vi "Test Li.vi"() -> ()   [LabVIEW 2026]
panel:
  out "XY Graph":cluster{dbl[], dbl[]}[](graph)
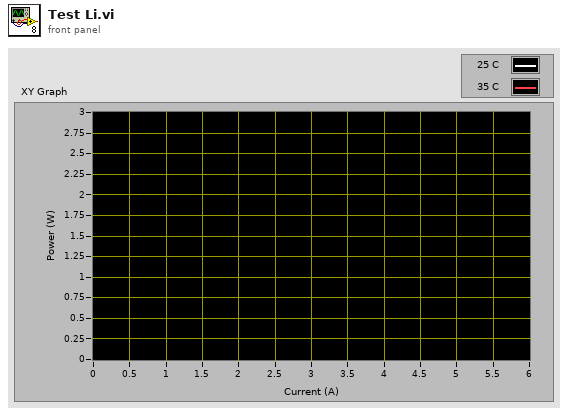
[diagram p1: front panel]
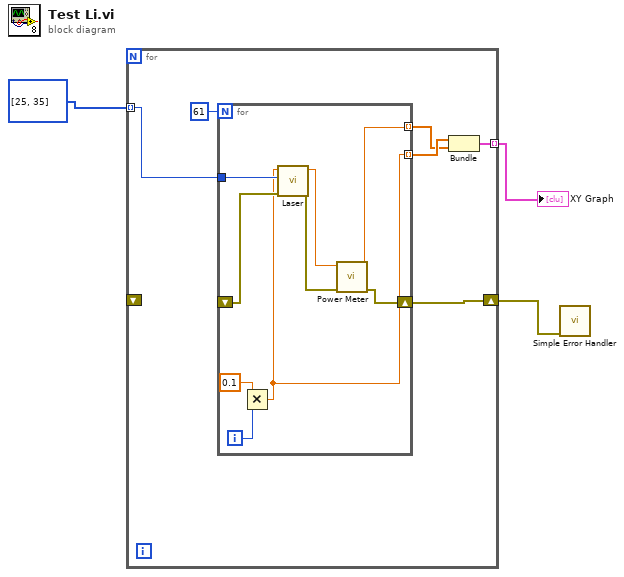
[diagram p0: block diagram]
diagram:
  n1 = for {
    tunnel: i32[] [25, 35] -> [w8] mode=indexing
    shift-right: [w7] -> w1
    shift-left: _ -> [_]
    tunnel: [w4] -> w2 mode=indexing
    n2 = for {
      N: 61 -> [_]
      tunnel: w8 -> [w16]
      shift-right: [w13] -> w7
      shift-left: _ -> [w12]
      tunnel: [w11] -> w5 mode=indexing
      tunnel: [w10] -> w6 mode=indexing
      i -> [w18]
      n3 = Multiply(x=0.1, y=w18) -> (x*y=w10:dbl)
      n4 = call "Laser.vi"("error in (no error)"=w12, "Temp (C)"=w16, "Current (A)"=w10) -> ("error out"=w14:errorcluster, "Power (W)"=w15:dbl)  [unwired: 6 in, 1 out]
      n5 = call "Power Meter.vi"("error in (no error)"=w14, "True Power (W)"=w15) -> ("error out"=w13:errorcluster, "Reading (W)"=w11:dbl)  [unwired: 8 in]
    }
    n6 = Bundle(w6, w5) -> (w4:cluster{dbl[], dbl[]})  [unwired: 1 in]
  }
  "XY Graph" <- w2
  n7 = call <vilib>:"Simple Error Handler.vi"("error in (no error)"=w1) -> ()  [unwired: 4 in, 5 out]
